vi "upload_ingest.video.vi"(4 "Properties":map{string, string}(c390), 6 "Labels":string[](array[string]), 7 "Time Stamp":timestamp format="%<%x %.3X>T", 8 "error in":errorcluster, 10 "File Path":path, 11 "Nominal Client in":refnum<class "Nominal Client.lvclass">) -> (0 "error out":errorcluster, 2 "videoRid":string, 3 "Nominal Client out":refnum<class "Nominal Client.lvclass">)   [LabVIEW 2020, in "Nominal Client.lvclass"]
doc: "Uploads a file to S3\nIngests video with common settings:\n - No TimeManifest (uses Start Timestamp and a scale factor of 1.\nNew Target: Name based on path name and timestamp"
uses:
  Nominal Client.lvclass
  datasources/dataset/dataset.lvclass
  nominal types/channelConfig/channelConfig.lvclass
  nominal types/timestampManifest/noManifest/noManifest.lvclass
  C:/code/labview-client/lv_src/nominal types/timestampManifest/timestampManifest/timestampManifest.lvclass
  datasources/target.video/target.video.lvclass
  C:/code/labview-client/lv_src/Nominal Client/datasources/target/target.lvclass
  datasources/s3/s3.lvclass
  C:/code/labview-client/lv_src/Nominal Client/datasources/source/source.lvclass
  datasources/source/create_s3.vi
  nominal types/timestampManifest/create.noManifest_scale_factor.vi
  datasources/target.video/create.new_video.vi
  ingest_video.vi
  Nominal Client.lvclass/Nominal Client.ctl
  datasources/target/target.lvclass
  datasources/source/source.lvclass
  nominal types/timestampManifest/timestampManifest.lvlib
  C:/code/labview-client/lv_src/Nominal Client/datasources/payload/payload.lvclass
  C:/code/labview-client/lv_src/nominal types/timestampManifest/noManifest/noManifest.lvclass
  C:/code/labview-client/lv_src/Nominal Client/datasources/target.video/target.video.lvclass
  C:/code/labview-client/lv_src/Nominal Client/datasources/s3/s3.lvclass
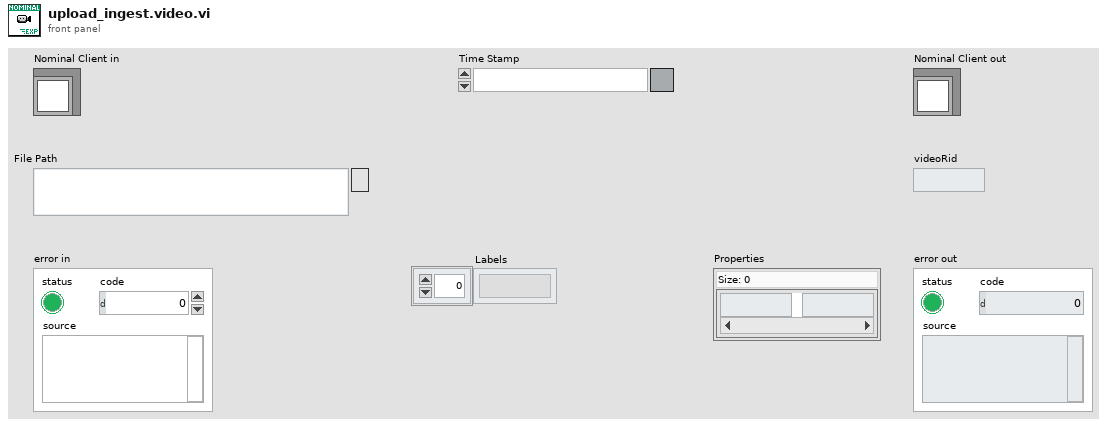
[diagram p1: front panel]
types:
  T1 = cluster{"dataset":refnum<class "dataset.lvclass">, "channelConfig":refnum<class "channelConfig.lvclass">}
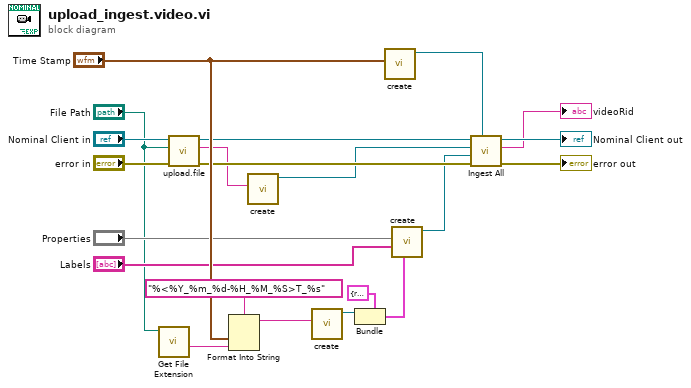
[diagram p0: block diagram]
diagram:
  n1 = call <vilib>:"Get File Extension.vi"("file"="File Path") -> ("filename without extension"=w3:string)  [unwired: 6 in, 4 out]
  n2 = call "upload.file.vi"("error in"="error in", "File"="File Path", "Nominal Client in"="Nominal Client in") -> ("error out"=w19:errorcluster, "Path to S3 File"=w17:string, "Nominal Client out"=w20:refnum<class "Nominal Client.lvclass">)  [unwired: 6 in]
  n3 = Format Into String(format string="%<%Y_%m_%d-%H_%M_%S>T_%s", "Time Stamp", w3) -> (resulting string=w2:string)  [unwired: 2 in, 1 out]
  n4 = call-poly "create.vi"("Path"=w17) -> ("source"=w16:refnum<class "s3.lvclass">)  [unwired: 10 in]
  n5 = call "create.vi"("Name"=w2) -> ("dataset"=w14:refnum<class "dataset.lvclass">)  [unwired: 10 in]
  n6 = Bundle(cluster=T1 {"dataset"=refnum, "channelConfig"=refnum} ("Optional"), "dataset"=w14) -> (w13:T1)  [unwired: 1 in]
  n7 = call-poly "create.vi"("startingTimestamp"="Time Stamp") -> ("Timestamp Manifest"=w1:refnum<class "noManifest.lvclass">)  [unwired: 10 in]
  n8 = call-poly "create.vi"("Optional"=w13, "Labels"="Labels", "Properties"="Properties") -> ("target video"=w18:refnum<class "target.video.lvclass">)  [unwired: 7 in, 1 out]
  n9 = call-poly "Ingest All.vi"("Timestamp Manifest"=w1, "error in"=w19, "Target"=w18, "Source"=w16, "Nominal Client in"=w20) -> ("error out"=→"error out":errorcluster, "videoRid"=→"videoRid":string, "Nominal Client out"=→"Nominal Client out":refnum<class "Nominal Client.lvclass">)  [unwired: 3 in, 1 out]
